vi "VIH HelpGen - Build Log Handler - CHM File.vi"(6 "cmd (nop)":T2(ring), 8 "error in":errorcluster, 9 "File Built":bool, 11 "File Path 1":path) -> (0 "error out":errorcluster, 2 "errors":i32, 3 "CHM status":T1)   [LabVIEW 2014]
doc: "::: VI Helpeks :::\nCopyright (c) 2000-2026 Konstantin Shifershteyn. All rights reserved."
panel:
  # "VI Helpeks\nCopyright (c) 2012-2026 Konstantin Shifershteyn"
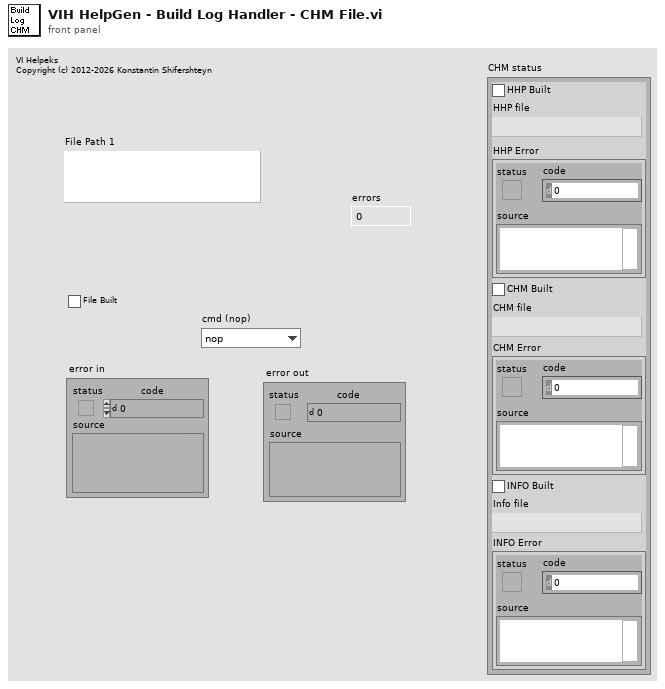
[diagram p1: front panel]
types:
  T1 = cluster{"HHP Built":bool, "HHP file":path, "HHP Error":errorcluster, "CHM Built":bool, "CHM file":path, "CHM Error":errorcluster, "INFO Built":bool, "Info file":path, "INFO Error":errorcluster}
  T2 = enum16{"nop", "Init", "Run-HHP", "Run-CHM", "Run-INFO"}
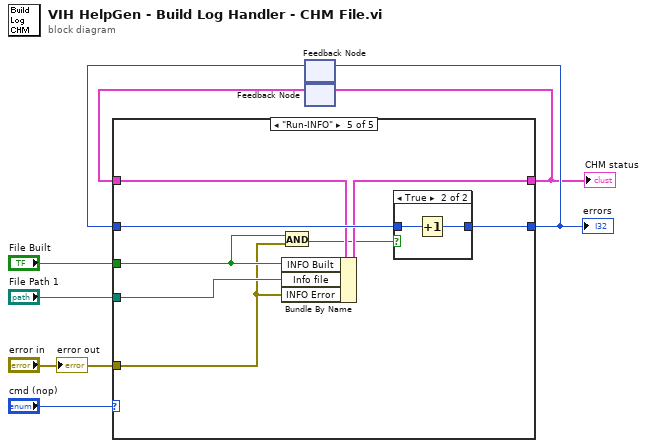
[diagram p0: block diagram]
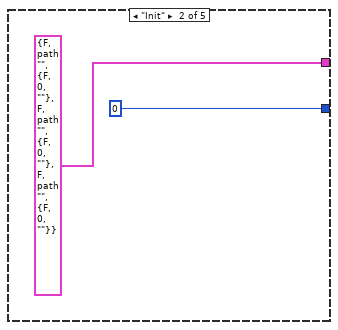
[diagram p3: hidden frame]
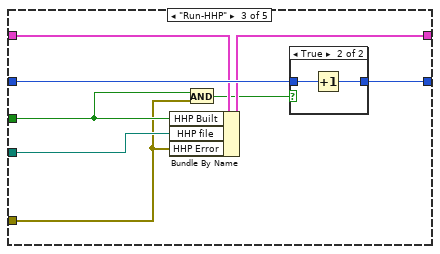
[diagram p4: hidden frame]
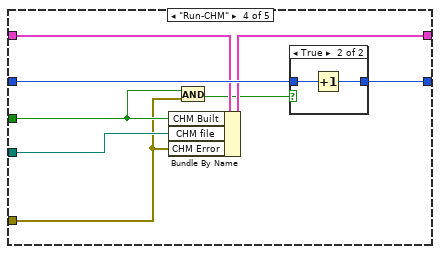
[diagram p6: hidden frame]
diagram:
  n1 = feedback #1() -> (w3:i32)  [unwired: 1 in]
  n2 = feedback #2() -> (w6:T1)  [unwired: 1 in]
  n3 = case shown="\"Run-INFO\"" "cmd (nop)" {
    tunnel: "File Path 1" -> [_ _ w16 w27 w38]
    tunnel: [w9 T1 {"HHP Built"=FALSE, "HHP file"=path "", "HHP Error"={"status"=FALSE, "code"=0, "source"=""}, "CHM Built"=FALSE, "CHM file"=path "", "CHM Error"={"status"=FALSE, "code"=0, "source"=""}, "INFO Built"=FALSE, "Info file"=path "", "INFO Error"={"status"=FALSE, "code"=0, "source"=""}} ("CHM status") w17 w28 w39] -> w1
    tunnel: w6 -> [w9 _ w18 w29 w40]
    tunnel: "error in" -> [_ _ w14 w25 w35]
    tunnel: [w10 0 w19 w30 w41] -> w4
    tunnel: w3 -> [w10 _ w20 w31 w42]
    tunnel: "File Built" -> [_ _ w15 w26 w36]
    frame "nop" {
    }
    frame "Init" {
    }
    frame "Run-HHP" {
      n4 = Bundle By Name(cluster=w18, "HHP Built"=w15, "HHP file"=w16, "HHP Error"=w14) -> (w17:T1)
      n5 = And(x=w15, y=w14) -> (x .and. y?=w13:bool)
      n6 = case shown="True" w13 {
        tunnel: w20 -> [w21 w23]
        tunnel: [w21 w22] -> w19
        frame False {
        }
        frame True {
          n7 = Increment(x=w23) -> (x+1=w22:i32)
        }
      }
    }
    frame "Run-CHM" {
      n8 = Bundle By Name(cluster=w29, "CHM Built"=w26, "CHM file"=w27, "CHM Error"=w25) -> (w28:T1)
      n9 = And(x=w26, y=w25) -> (x .and. y?=w24:bool)
      n10 = case shown="True" w24 {
        tunnel: w31 -> [w32 w34]
        tunnel: [w32 w33] -> w30
        frame False {
        }
        frame True {
          n11 = Increment(x=w34) -> (x+1=w33:i32)
        }
      }
    }
    frame "Run-INFO" {
      n12 = And(x=w36, y=w35) -> (x .and. y?=w37:bool)
      n13 = Bundle By Name(cluster=w40, "INFO Built"=w36, "Info file"=w38, "INFO Error"=w35) -> (w39:T1)
      n14 = case shown="True" w37 {
        tunnel: w42 -> [w43 w45]
        tunnel: [w43 w44] -> w41
        frame False {
        }
        frame True {
          n15 = Increment(x=w45) -> (x+1=w44:i32)
        }
      }
    }
  }
  "errors" <- w4
  "CHM status" <- w1
  n16 = feedback-in #1(w4) -> ()
  n17 = feedback-in #2(w1) -> ()
  "error out" <- "error in"
